vi "Orca Flash Engine.vi"(0 "Notifier Name":string, 11 "Camera ID":string[](array[string])) -> ()   [LabVIEW 2021]
uses:
  Orca Flash Controls/Orca Flash Parameters.ctl
  Orca Flash Controls/Orca Flash Parameter List.ctl
  Orca Flash Controls/Orca Flash ROI.ctl
  Orca Flash Controls/Orca Flash Notifier Element.ctl
  Orca Flash Controls/Orca Flash Actions.ctl
  <vilib>/vision/Image Controls.llb/IMAQ Image.ctl
  Camera Controls/Camera IMAQ Key Info.ctl
panel:
  out "bead collection":bool
  in  "Orca Flash ROI":T1
  in  "Use Display Module":bool
  in  "Sensor Mode":enum32{"Area", "Progressive"}(radio)
  in  "Number of lines":dbl=8.0
  in  "Internal Line Interval Setpoint":dbl=0.001
  in  "Get Parameter":bool
  in  "Set Parameter":bool
  in  "Get ROI":bool
  in  "Set ROI":bool
  in  "sCMOS Parameter":T2={"Value"=0.0, "Orca Flash Parameters"=2049184} {"Orca Flash Parameters" items=["SENSOR MODE"=4212128, "READOUT SPEED"=4211872, "READOUT DIRECTION"=4211904, "TRIGGER GLOBAL EXPOSURE"=2049680, "TRIGGER DELAY"=1066480, "SYNC READOUT SYSTEM BLANK"=1066528, "SENSOR COOLER"=2115248, "SENSOR COOLER STATUS"=2115280, "EXPOSURE TIME"=2049184, "DEFECT CORRECT MODE"=4670368, "BINNING"=4215968, "INTERNAL FRAME RATE"=4225952, "INTERNAL FRAME INTERVAL"=4225968, "INTERNAL LINE SPEED"=4226000, "INTERNAL LINE INTERVAL"=4226016, "IMAGE PIXEL TYPE"=4343296, "NUMBER OF OUTPUT TRIGGER CONNECTOR"=1852320, "OUTPUT TRIGGER SOURCE[0]"=1852576, "OUTPUT TRIGGER SOURCE[1]"=1852832, "OUTPUT TRIGGER SOURCE[2]"=1853088, "OUTPUT TRIGGER POLARITY[0]"=1852592, "OUTPUT TRIGGER POLARITY[1]"=1852848, "OUTPUT TRIGGER POLARITY[2]"=1853104, "OUTPUT TRIGGER ACTIVE[0]"=1852608, "OUTPUT TRIGGER ACTIVE[1]"=1852864, "OUTPUT TRIGGER ACTIVE[2]"=1853120, "OUTPUT TRIGGER DELAY[0]"=1852624, "OUTPUT TRIGGER DELAY[1]"=1852880, "OUTPUT TRIGGER DELAY[2]"=1853136, "OUTPUT TRIGGER PERIOD[0]"=1852640, "OUTPUT TRIGGER PERIOD[1]"=1852896, "OUTPUT TRIGGER PERIOD[2]"=1853152, "OUTPUT TRIGGER KIND[0]"=1852656, "OUTPUT TRIGGER KIND[1]"=1852912, "OUTPUT TRIGGER KIND[2]"=1853168, "OUTPUT TRIGGER PRE HSYNC COUNT"=1852704]}
  in  "# of frames":i32=100
  in  "Path":path
  in  "RECORD":bool
  in  "PREVIEW":bool
  out "Acquisition Loop":i32
  in  "QUIT":bool
  out "Acquisition Frame":i32
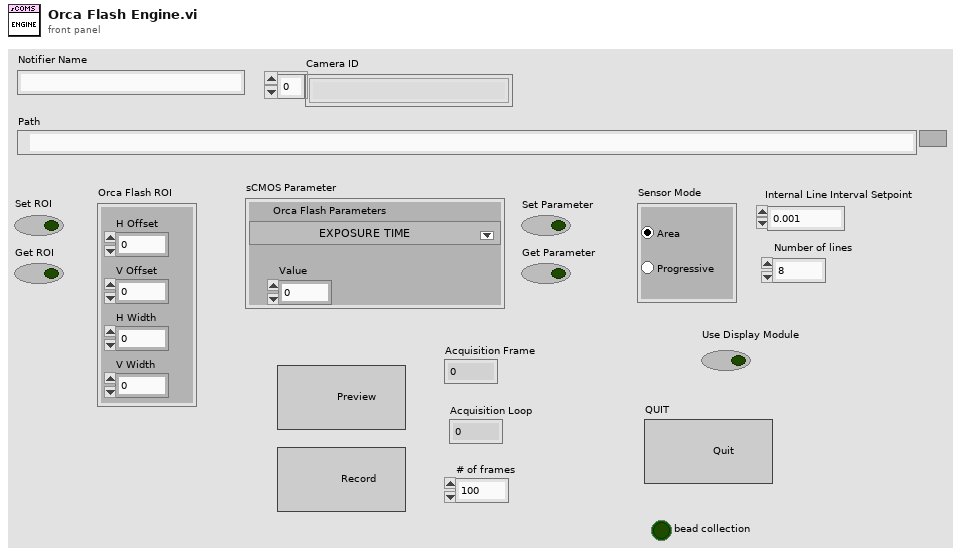
[diagram p1: front panel]
types:
  T1 = typedef "Orca Flash ROI.ctl" = cluster{"H Offset":i32, "V Offset":i32, "H Width":i32, "V Width":i32}
  T2 = typedef "Orca Flash Parameters.ctl" = cluster{"Value":dbl, "Orca Flash Parameters":T3}
  T3 = typedef "Orca Flash Parameter List.ctl" = u32
  T4 = typedef "Camera IMAQ Key Info.ctl" = cluster{"Frame":u32, "Sensor Height":i32, "Sensor Width":i32, "ROI Height":i32, "ROI Width":i32, "ROI Enable?":bool, "Bit per Pixel":u8}
  T5 = typedef "Image Type" = u32
  T6 = typedef "Orca Flash Notifier Element.ctl" = cluster{"Camera Actions":T7, "Received?":bool, "Running?":bool, "sCMOS Parameter":T2, "sCMOS ROI":T1, "Save Path":path, "# of frames":u32, "Image Ref":T8, "Trigger?":bool, "bead collection":bool}
  T7 = typedef "Orca Flash Actions.ctl" = enum16{"IDLE", "PREVIEW", "RECORD", "Send Trigger", "SOFT TRIGGER", "Record Settings", "SETPARAM", "GETPARAM", "SETROI", "GETROI", "PROGRESSIVE MODE", "AREA MODE", "STATUS", "QUIT"}
  T8 = typedef "IMAQ Image.ctl" = refnum<image>
  T9 = enum32{"Invalid", "Standard", "Closed", "Hidden", "Minimized", "Maximized"}
  T10 = cluster{"Horizontal Offset":i32, "Vertical Offset":i32, "Horizontal Size":i32, "Vertical Size":i32}
  T11 = typedef "LVMinMaxIncTypeDef.ctl" = cluster{"Minimum":dbl, "Maximum":dbl, "Increment":dbl}
  T12 = cluster{"H Offset":cluster{"Value":i32, "Limits":T11}, "V Offset":cluster{"Value":i32, "Limits":T11}, "H Size":cluster{"Value":i32, "Limits":T11}, "V Size":cluster{"Value":i32, "Limits":T11}}
  T13 = cluster{"Input Trigger Mode":u32, "Input Trigger Polarity":u32, "Times":u32, "Delay":dbl}
  T14 = cluster{"Output Trigger Period":dbl, "Delay":dbl, "Source":u32}
  T15 = cluster{"Output Trigger Mode":u32, "Output Trigger Polarity":u32}
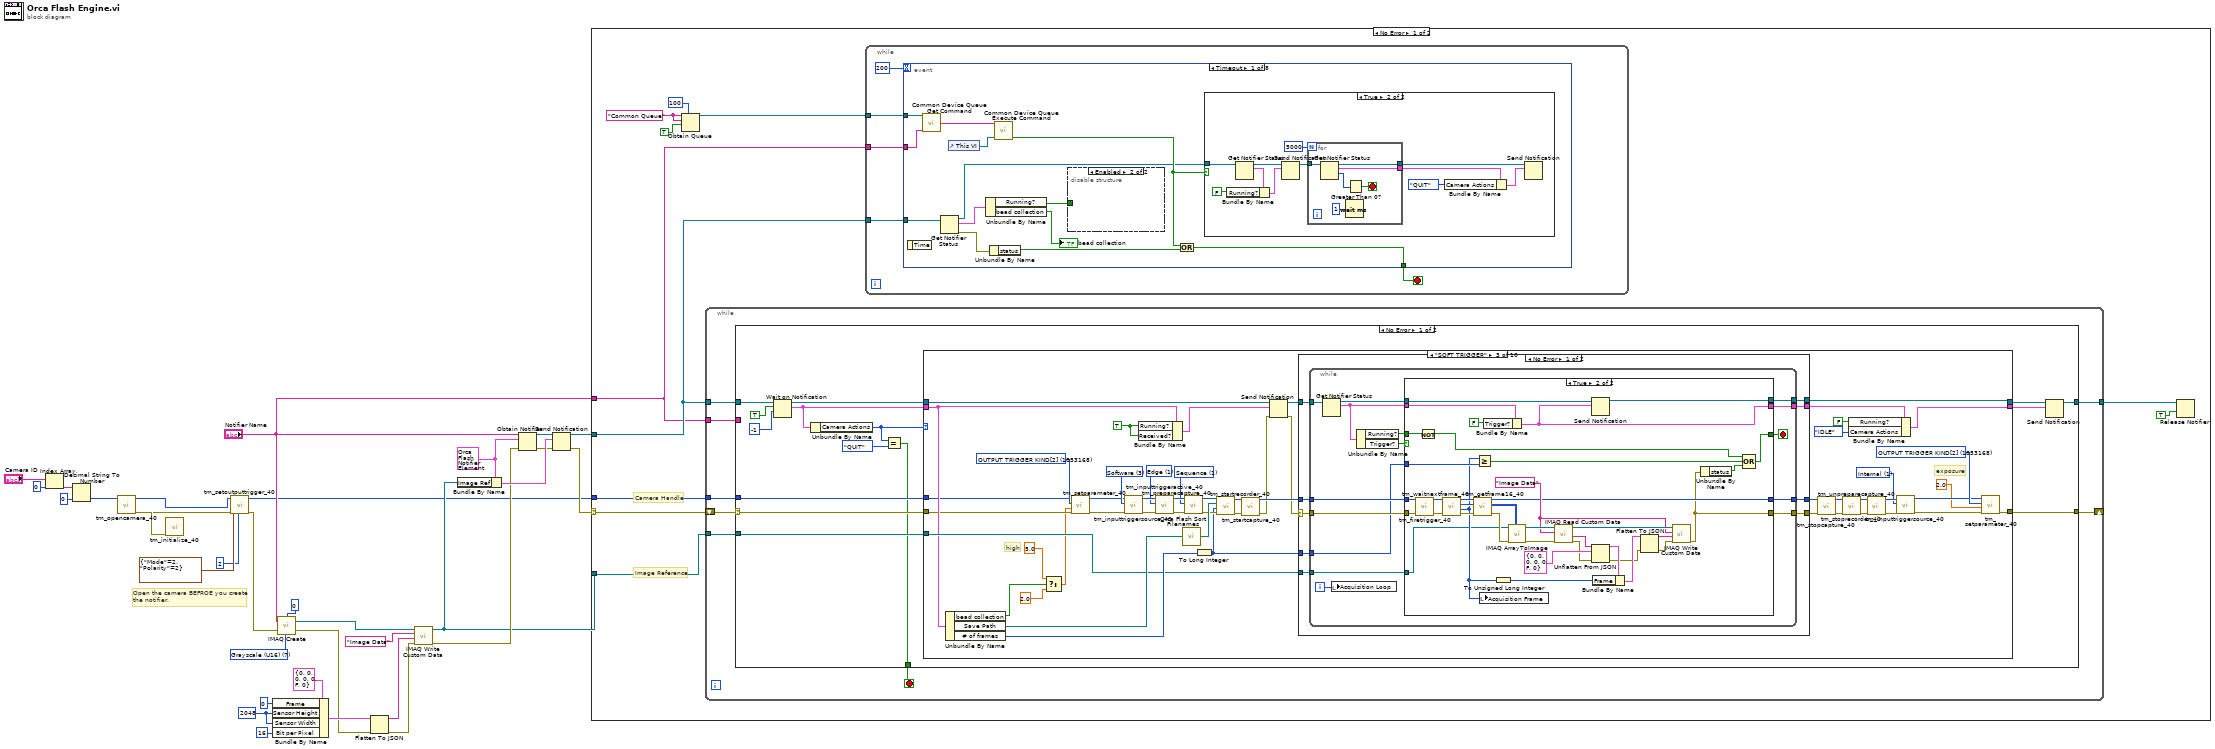
[diagram p0: block diagram]
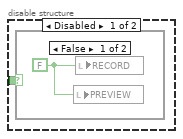
[diagram p2: hidden frame]
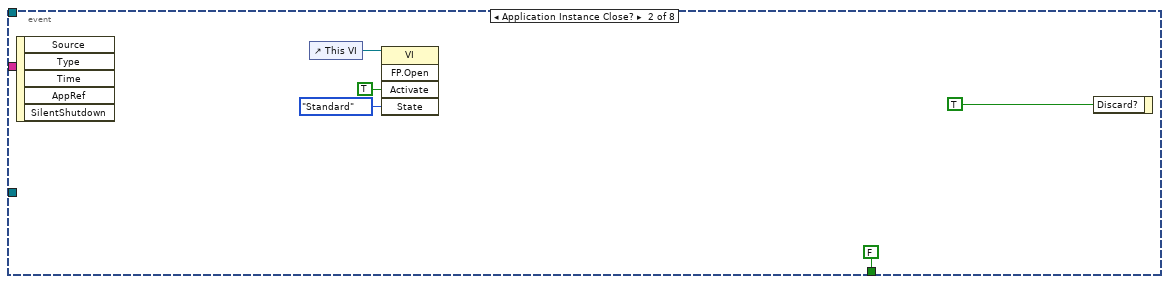
[diagram p5: hidden frame]
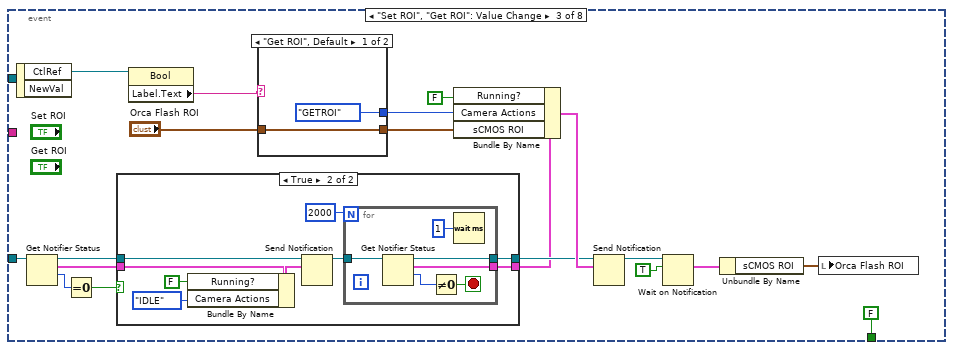
[diagram p6: hidden frame]
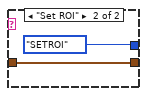
[diagram p8: hidden frame]
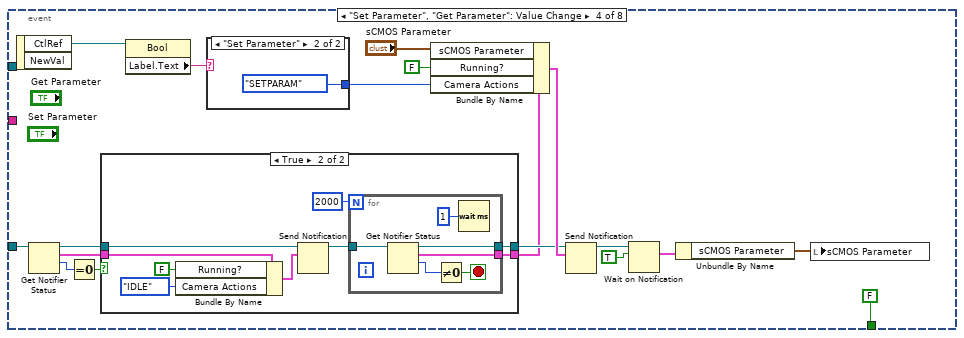
[diagram p9: hidden frame]
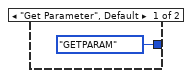
[diagram p11: hidden frame]
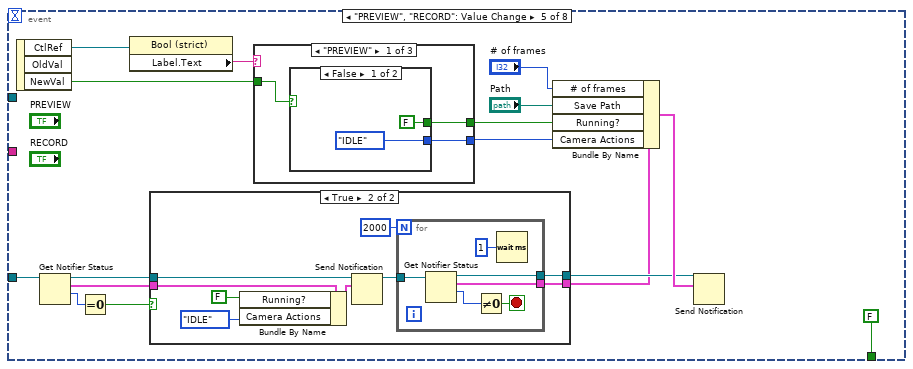
[diagram p12: hidden frame]
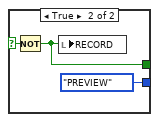
[diagram p13: hidden frame]
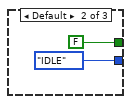
[diagram p14: hidden frame]
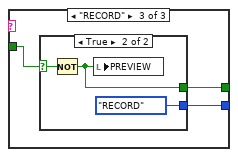
[diagram p15: hidden frame]
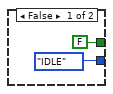
[diagram p16: hidden frame]
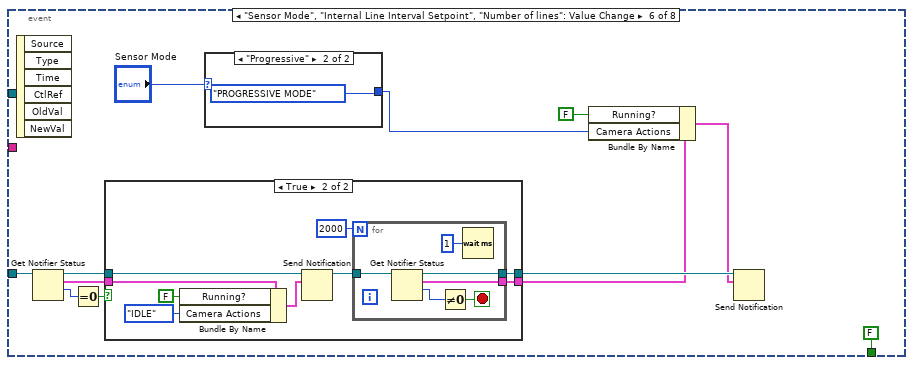
[diagram p18: hidden frame]
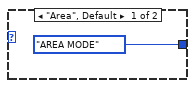
[diagram p19: hidden frame]
diagram:
  w18 = 2048 ("Sensor Height")
  w14 = T5 7 items=["Grayscale (U8)", "Grayscale (I16)", "Grayscale (SGL)", "Complex (CSG)", "RGB (U32)", "HSL (U32)", "RGB (U64)", "Grayscale (U16)"] ("Image Type")
  w28 = T6 {"Camera Actions"=enum."IDLE", "Received?"=FALSE, "Running?"=FALSE, "sCMOS Parameter"={"Value"=0.0, "Orca Flash Parameters"=0}, "sCMOS ROI"={"H Offset"=0, "V Offset"=0, "H Width"=0, "V Width"=0}, "Save Path"=path "", "# of frames"=1, "Image Ref"=refnum, "Trigger?"=FALSE, "bead collection"=FALSE} ("Camera Cluster")
  # "Open the camera BEFROE you create\nthe notifier."
  n1 = Index Array(array="Camera ID", index=0) -> (element=w31:string)
  n2 = Decimal String To Number(string=w31, default (0L)=u32 0 ("default (0 I32)")) -> (number=w24:u32)  [unwired: 1 in, 1 out]
  n3 = call <userlib>:"tm_initialize_40.vi"() -> ("error out"=w25:errorcluster)  [unwired: 8 in, 3 out]
  n4 = call <userlib>:"tm_opencamera_40.vi"("error in (no error)"=w25, "Camera Index"=w24) -> ("error out"=w4:errorcluster, "Handle out"=w3:u32)  [unwired: 7 in, 1 out]
  n5 = call <userlib>:"tm_setoutputtrigger_40.vi"("Port"=2, "error in (no error)"=w4, "Type"=cluster{"Mode":u32, "Polarity":u32} {"Mode"=2, "Polarity"=2}, "Handle in"=w3) -> ("error out"=w6:errorcluster, "Handle out"=w5:u32)  [unwired: 6 in]
  n6 = Bundle By Name(cluster=T4 {"Frame"=0, "Sensor Height"=0, "Sensor Width"=0, "ROI Height"=0, "ROI Width"=0, "ROI Enable?"=FALSE, "Bit per Pixel"=0} ("Camera IMAQ Key Info"), "Frame"=u32 0, "Sensor Height"=w18, "Sensor Width"=w18, "Bit per Pixel"=u8 16) -> (w21:T4)
  n7 = call "IMAQ Create"("Border Size"=0, "Image Name"="Notifier Name", "Image Type"=w14, "error in (no error)"=w6) -> ("New Image"=w16:T8, "error out"=w13:errorcluster)  [unwired: 1 in]
  n8 = Flatten To JSON(anything=w21, error in (no error)=w13) -> (JSON string=w22:string, 11:w12:errorcluster)  [unwired: 1 in]
  n9 = call "IMAQ Write Custom Data"("error in (no error)"=w12, "Custom Data In"=w22, "Key"="Image Data", "Image"=w16) -> ("error out"=w11:errorcluster, "Image Out"=w8:T8)  [unwired: 6 in]
  n10 = Bundle By Name(cluster=w28, "Image Ref"=w8) -> (w29:T6)
  n11 = Obtain Notifier(name (unnamed)="Notifier Name", notification data type=w28, error in (no error)=w11) -> (notifier out=w27:refnum<notifier>, error out=w26:errorcluster)  [unwired: 1 in, 1 out]
  n12 = Send Notification(notification=w29, notifier=w27, error in (no error)=w26) -> (notifier out=w10:refnum<notifier>, error out=w7:errorcluster)
  n13 = case shown="No Error" w7 {
    selector: w7 -> [w39 w760]
    tunnel: w10 -> [w37 w753]
    tunnel: "Notifier Name" -> [w34 w750]
    tunnel: w8 -> [w40 _]
    tunnel: w5 -> [w38 _]
    frame No Error {
      w44 = "Common Queue" ("Unique Notifier Name")
      # "Image Reference"
      # "Camera Handle"
      n14 = Obtain Queue(max queue size (-1, unlimited)=100, name (unnamed)=w44, element data type=w44, create if not found? (T)=TRUE) -> (queue out=w41:refnum<queue>)  [unwired: 1 in, 2 out]
      n15 = while {
        tunnel: w37 -> [w319]
        tunnel: w40 -> [w318]
        shift-right: [w316] -> _
        shift-left: w39 -> [w315]
        tunnel: w38 -> [w317]
        tunnel: [w314] -> w35
        tunnel: w34 -> [w312]
        stop <- w313 stop-if-true
        n16 = case shown="No Error" w315 {
          selector: w315 -> [w324 w741]
          tunnel: w319 -> [w334 w749]
          tunnel: w318 -> [w333 _]
          tunnel: [w323 w749] -> w314
          tunnel: w317 -> [w326 _]
          tunnel: [w325 errorcluster {"status"=FALSE, "code"=0, "source"=""} ("error out")] -> w316
          tunnel: [w320 FALSE] -> w313
          tunnel: w312 -> [_ w740]
          frame No Error {
            n17 = Wait on Notification(notifier=w334, ignore previous (F)=TRUE, timeout in ms (-1)=-1) -> (notifier out=w329:refnum<notifier>, notification=w328:T6)  [unwired: 1 in, 2 out]
            n18 = Unbundle By Name(w328) -> ("Camera Actions"=w322:T7)
            n19 = Equal?(x=w322, y=Orca_Flash_Actions."QUIT") -> (x = y?=w320:bool)
            n20 = case shown="\"SOFT TRIGGER\"" w322 {
              selector: w322 -> [_ w358 _ _ _ _ _ _ _ _]
              tunnel: w326 -> [_ w353 w466 w581 w597 w610 w644 w655 w676 w730]
              tunnel: w324 -> [w339 w350 w465 w582 w596 w609 w643 w654 w675 w729]
              tunnel: [w339 w344 w459 w580 w592 w608 w636 w653 w663 w719] -> w325
              tunnel: w329 -> [w338 w384 w472 w588 w601 w611 w645 w660 w690 w739]
              tunnel: w333 -> [_ w355 w477 w583 _ _ w612 _ _ _]
              tunnel: w328 -> [w336 w375 w473 w586 w595 w606 w639 w657 w687 w726]
              tunnel: [w338 w376 w476 w588 w601 w611 w645 w660 w690 w739] -> w330
              tunnel: [w335 w371 w478 w585 w600 w602 w638 w656 w686 w725] -> w327
              frame "IDLE", Default {
                w337 = FALSE ("Running?")
                n21 = Bundle By Name(cluster=w336, "Received?"=w337, "Running?"=w337) -> (w335:T6)
              }
              frame "PREVIEW", "RECORD" {
                w348 = T3 1853168 items=["SENSOR MODE"=4212128, "READOUT SPEED"=4211872, "READOUT DIRECTION"=4211904, "TRIGGER GLOBAL EXPOSURE"=2049680, "TRIGGER DELAY"=1066480, "SYNC READOUT SYSTEM BLANK"=1066528, "SENSOR COOLER"=2115248, "SENSOR COOLER STATUS"=2115280, "EXPOSURE TIME"=2049184, "DEFECT CORRECT MODE"=4670368, "BINNING"=4215968, "INTERNAL FRAME RATE"=4225952, "INTERNAL FRAME INTERVAL"=4225968, "INTERNAL LINE SPEED"=4226000, "INTERNAL LINE INTERVAL"=4226016, "IMAGE PIXEL TYPE"=4343296, "NUMBER OF OUTPUT TRIGGER CONNECTOR"=1852320, "OUTPUT TRIGGER SOURCE[0]"=1852576, "OUTPUT TRIGGER SOURCE[1]"=1852832, "OUTPUT TRIGGER SOURCE[2]"=1853088, "OUTPUT TRIGGER POLARITY[0]"=1852592, "OUTPUT TRIGGER POLARITY[1]"=1852848, "OUTPUT TRIGGER POLARITY[2]"=1853104, "OUTPUT TRIGGER ACTIVE[0]"=1852608, "OUTPUT TRIGGER ACTIVE[1]"=1852864, "OUTPUT TRIGGER ACTIVE[2]"=1853120, "OUTPUT TRIGGER DELAY[0]"=1852624, "OUTPUT TRIGGER DELAY[1]"=1852880, "OUTPUT TRIGGER DELAY[2]"=1853136, "OUTPUT TRIGGER PERIOD[0]"=1852640, "OUTPUT TRIGGER PERIOD[1]"=1852896, "OUTPUT TRIGGER PERIOD[2]"=1853152, "OUTPUT TRIGGER KIND[0]"=1852656, "OUTPUT TRIGGER KIND[1]"=1852912, "OUTPUT TRIGGER KIND[2]"=1853168, "OUTPUT TRIGGER PRE HSYNC COUNT"=1852704] ("sCMOS Parameter.Orca Flash Parameters")
                w351 = T3 1853168 items=["SENSOR MODE"=4212128, "READOUT SPEED"=4211872, "READOUT DIRECTION"=4211904, "TRIGGER GLOBAL EXPOSURE"=2049680, "TRIGGER DELAY"=1066480, "SYNC READOUT SYSTEM BLANK"=1066528, "SENSOR COOLER"=2115248, "SENSOR COOLER STATUS"=2115280, "EXPOSURE TIME"=2049184, "DEFECT CORRECT MODE"=4670368, "BINNING"=4215968, "INTERNAL FRAME RATE"=4225952, "INTERNAL FRAME INTERVAL"=4225968, "INTERNAL LINE SPEED"=4226000, "INTERNAL LINE INTERVAL"=4226016, "IMAGE PIXEL TYPE"=4343296, "NUMBER OF OUTPUT TRIGGER CONNECTOR"=1852320, "OUTPUT TRIGGER SOURCE[0]"=1852576, "OUTPUT TRIGGER SOURCE[1]"=1852832, "OUTPUT TRIGGER SOURCE[2]"=1853088, "OUTPUT TRIGGER POLARITY[0]"=1852592, "OUTPUT TRIGGER POLARITY[1]"=1852848, "OUTPUT TRIGGER POLARITY[2]"=1853104, "OUTPUT TRIGGER ACTIVE[0]"=1852608, "OUTPUT TRIGGER ACTIVE[1]"=1852864, "OUTPUT TRIGGER ACTIVE[2]"=1853120, "OUTPUT TRIGGER DELAY[0]"=1852624, "OUTPUT TRIGGER DELAY[1]"=1852880, "OUTPUT TRIGGER DELAY[2]"=1853136, "OUTPUT TRIGGER PERIOD[0]"=1852640, "OUTPUT TRIGGER PERIOD[1]"=1852896, "OUTPUT TRIGGER PERIOD[2]"=1853152, "OUTPUT TRIGGER KIND[0]"=1852656, "OUTPUT TRIGGER KIND[1]"=1852912, "OUTPUT TRIGGER KIND[2]"=1853168, "OUTPUT TRIGGER PRE HSYNC COUNT"=1852704] ("sCMOS Parameter.Orca Flash Parameters")
                w356 = TRUE ("Running?")
                w381 = 1 items=["Snap", "Sequence"] ("Capture mode")
                # "exposure"
                # "high"
                n22 = Unbundle By Name(w375) -> ("bead collection"=w340:bool, "# of frames"=w364:u32, "Save Path"=w354:path)
                n23 = Select(t=5.0 ("Value in"), s=w340, f=2.0 ("Value in")) -> (s? t:f=w341:dbl)
                n24 = call <userlib>:"tm_setparameter_40.vi"("error in (no error)"=w350, "Value in"=w341, "Parameter"=w351, "Handle in"=w353) -> ("error out"=w349:errorcluster, "Handle out"=w352:u32)  [unwired: 6 in]
                n25 = Equal?(x=w358, y=Orca_Flash_Actions."RECORD") -> (x = y?=w357:bool)
                n26 = call <userlib>:"tm_preparecapture_40.vi"("error in (no error)"=w349, "Capture mode"=w381, "Handle in"=w352) -> ("error out"=w383:errorcluster, "Handle out"=w382:u32)  [unwired: 5 in, 2 out]
                n27 = To Long Integer(number=w364) -> (32bit integer=w362:i32)
                n28 = case shown="True" w357 {
                  tunnel: w383 -> [w386 w393]
                  tunnel: w382 -> [w385 w392]
                  tunnel: [w385 w391] -> w370
                  tunnel: [w386 w390] -> w368
                  tunnel: w362 -> [_ w389]
                  tunnel: w354 -> [_ w388]
                  frame False {
                  }
                  frame True {
                    n29 = call "Orca Flash Sort Filenames.vi"("Requested File Path"=w388) -> ("Resulting File Path"=w387:path)  [unwired: 14 in]
                    n30 = call <userlib>:"tm_startrecorder_40.vi"("error in (no error)"=w393, "frames"=w389, "File"=w387, "Handle in"=w392) -> ("error out"=w390:errorcluster, "Handle out"=w391:u32)  [unwired: 6 in]
                  }
                }
                n31 = Bundle By Name(cluster=w375, "Running?"=w356, "Received?"=w356) -> (w374:T6)
                n32 = call <userlib>:"tm_startcapture_40.vi"("error in (no error)"=w368, "Handle in"=w370) -> ("error out"=w361:errorcluster, "Handle out"=w369:u32)  [unwired: 8 in]
                n33 = Send Notification(notification=w374, notifier=w384, error in (no error)=w361) -> (notifier out=w377:refnum<notifier>, error out=w360:errorcluster)
                n34 = case shown="No Error" w360 {
                  selector: w360 -> [w401 w451]
                  tunnel: [w409 w452] -> w380
                  tunnel: w377 -> [w408 w453]
                  tunnel: w355 -> [w407 _]
                  tunnel: [w406 w450] -> w376
                  tunnel: [w405 w449] -> w373
                  tunnel: w369 -> [w404 w452]
                  tunnel: [w403 w451] -> w367
                  tunnel: w362 -> [w402 _]
                  tunnel: w357 -> [w400 _]
                  frame No Error {
                    n35 = while {
                      tunnel: w402 -> [w437]
                      tunnel: w408 -> [w440]
                      tunnel: [w439] -> w406
                      tunnel: w407 -> [w436]
                      tunnel: [w434] -> w405
                      tunnel: w401 -> [w443]
                      tunnel: [w411] -> w403
                      tunnel: w404 -> [w444]
                      tunnel: [w432] -> w409
                      tunnel: w400 -> [w410]
                      i -> [w438]
                      stop <- w441 stop-if-true
                      w417 = "Image Data" ("Key")
                      n36 = call <userlib>:"tm_waitnextframe_40.vi"("error in (no error)"=w443, "Handle in"=w444) -> ("error out"=w428:errorcluster, "Frame Count"=w426:i32, "Frame Index"=w431:i32, "Handle out"=w442:u32)  [unwired: 6 in]
                      "Acquisition Frame" <- w426
                      n37 = call <userlib>:"tm_getframe16_40.vi"("error in (no error)"=w428, "Frame Index"=w431, "Handle in"=w442) -> ("error out"=w416:errorcluster, "Data"=w427:u16[][], "Handle out"=w432:u32)  [unwired: 5 in, 1 out]
                      n38 = case shown="True" w410 {
                        selector: w410 -> [w445 _]
                        tunnel: w437 -> [_ w448]
                        tunnel: [w445 w447] -> w429
                        tunnel: w426 -> [_ w446]
                        frame False {
                        }
                        frame True {
                          n39 = Greater Or Equal?(x=w446, y=w448) -> (x >= y?=w447:bool)
                        }
                      }
                      n40 = To Unsigned Long Integer(number=w426) -> (unsigned 32bit integer=w420:u32)
                      n41 = call "IMAQ ArrayToImage"("Image Pixels (U16)"=w427, "error in (no error)"=w416, "Image"=w436) -> ("error out"=w415:errorcluster, "Image Out"=w425:T8)  [unwired: 7 in]
                      n42 = call "IMAQ Read Custom Data"("error in (no error)"=w415, "Key"=w417, "Image"=w425) -> ("error out"=w414:errorcluster, "Custom Data Out"=w422:string, "Image (duplicate)"=w424:T8)  [unwired: 6 in]
                      n43 = Unflatten From JSON(JSON string=w422, type and defaults=T4 {"Frame"=0, "Sensor Height"=0, "Sensor Width"=0, "ROI Height"=0, "ROI Width"=0, "ROI Enable?"=FALSE, "Bit per Pixel"=0} ("Camera IMAQ Key Info"), error in (no error)=w414) -> (value=w421:T4, error out=w413:errorcluster)  [unwired: 4 in]
                      n44 = Bundle By Name(cluster=w421, "Frame"=w420) -> (w419:T4)
                      n45 = Get Notifier Status(notifier=w440) -> (notifier out=w439:refnum<notifier>, current notification=w434:T6)  [unwired: 1 in, 3 out]
                      n46 = Flatten To JSON(anything=w419, error in (no error)=w413) -> (JSON string=w418:string, 11:w412:errorcluster)  [unwired: 1 in]
                      n47 = Unbundle By Name(w434) -> ("Running?"=w435:bool)
                      n48 = call "IMAQ Write Custom Data"("error in (no error)"=w412, "Custom Data In"=w418, "Key"=w417, "Image"=w424) -> ("error out"=w411:errorcluster)  [unwired: 6 in, 1 out]
                      n49 = Unbundle By Name(w411) -> ("status"=w430:bool)
                      n50 = Not(x=w435) -> (.not. x?=w433:bool)
                      n51 = Compound Arithmetic op=OR(w433, w429, w430) -> (w441:bool)
                      "Acquisition Loop" <- w438
                    }
                  }
                  frame Error {
                    n52 = Get Notifier Status(notifier=w453) -> (notifier out=w450:refnum<notifier>, current notification=w449:T6)  [unwired: 1 in, 3 out]
                  }
                }
                n53 = call <userlib>:"tm_stopcapture_40.vi"("error in (no error)"=w367, "Handle in"=w380) -> ("error out"=w366:errorcluster, "Handle out"=w379:u32)  [unwired: 8 in]
                n54 = case shown="True" w357 {
                  tunnel: w379 -> [w395 w399]
                  tunnel: [w395 w398] -> w378
                  tunnel: w366 -> [w394 w397]
                  tunnel: [w394 w396] -> w365
                  frame False {
                  }
                  frame True {
                    n55 = call <userlib>:"tm_stoprecorder_40.vi"("error in (no error)"=w397, "Handle in"=w399) -> ("error out"=w396:errorcluster, "Handle out"=w398:u32)  [unwired: 8 in]
                  }
                }
                n56 = Bundle By Name(cluster=w373, "Running?"=FALSE, "Camera Actions"=Orca_Flash_Actions."IDLE") -> (w371:T6)
                n57 = call <userlib>:"tm_unpreparecapture_40.vi"("error in (no error)"=w365, "Handle in"=w378) -> ("error out"=w345:errorcluster, "Handle out"=w346:u32)  [unwired: 8 in]
                n58 = call <userlib>:"tm_setparameter_40.vi"("error in (no error)"=w345, "Value in"=2.0, "Parameter"=w348, "Handle in"=w346) -> ("error out"=w344:errorcluster)  [unwired: 6 in, 1 out]
              }
              frame "SOFT TRIGGER" {
                w462 = T3 1853168 items=["SENSOR MODE"=4212128, "READOUT SPEED"=4211872, "READOUT DIRECTION"=4211904, "TRIGGER GLOBAL EXPOSURE"=2049680, "TRIGGER DELAY"=1066480, "SYNC READOUT SYSTEM BLANK"=1066528, "SENSOR COOLER"=2115248, "SENSOR COOLER STATUS"=2115280, "EXPOSURE TIME"=2049184, "DEFECT CORRECT MODE"=4670368, "BINNING"=4215968, "INTERNAL FRAME RATE"=4225952, "INTERNAL FRAME INTERVAL"=4225968, "INTERNAL LINE SPEED"=4226000, "INTERNAL LINE INTERVAL"=4226016, "IMAGE PIXEL TYPE"=4343296, "NUMBER OF OUTPUT TRIGGER CONNECTOR"=1852320, "OUTPUT TRIGGER SOURCE[0]"=1852576, "OUTPUT TRIGGER SOURCE[1]"=1852832, "OUTPUT TRIGGER SOURCE[2]"=1853088, "OUTPUT TRIGGER POLARITY[0]"=1852592, "OUTPUT TRIGGER POLARITY[1]"=1852848, "OUTPUT TRIGGER POLARITY[2]"=1853104, "OUTPUT TRIGGER ACTIVE[0]"=1852608, "OUTPUT TRIGGER ACTIVE[1]"=1852864, "OUTPUT TRIGGER ACTIVE[2]"=1853120, "OUTPUT TRIGGER DELAY[0]"=1852624, "OUTPUT TRIGGER DELAY[1]"=1852880, "OUTPUT TRIGGER DELAY[2]"=1853136, "OUTPUT TRIGGER PERIOD[0]"=1852640, "OUTPUT TRIGGER PERIOD[1]"=1852896, "OUTPUT TRIGGER PERIOD[2]"=1853152, "OUTPUT TRIGGER KIND[0]"=1852656, "OUTPUT TRIGGER KIND[1]"=1852912, "OUTPUT TRIGGER KIND[2]"=1853168, "OUTPUT TRIGGER PRE HSYNC COUNT"=1852704] ("sCMOS Parameter.Orca Flash Parameters")
                w467 = T3 1853168 items=["SENSOR MODE"=4212128, "READOUT SPEED"=4211872, "READOUT DIRECTION"=4211904, "TRIGGER GLOBAL EXPOSURE"=2049680, "TRIGGER DELAY"=1066480, "SYNC READOUT SYSTEM BLANK"=1066528, "SENSOR COOLER"=2115248, "SENSOR COOLER STATUS"=2115280, "EXPOSURE TIME"=2049184, "DEFECT CORRECT MODE"=4670368, "BINNING"=4215968, "INTERNAL FRAME RATE"=4225952, "INTERNAL FRAME INTERVAL"=4225968, "INTERNAL LINE SPEED"=4226000, "INTERNAL LINE INTERVAL"=4226016, "IMAGE PIXEL TYPE"=4343296, "NUMBER OF OUTPUT TRIGGER CONNECTOR"=1852320, "OUTPUT TRIGGER SOURCE[0]"=1852576, "OUTPUT TRIGGER SOURCE[1]"=1852832, "OUTPUT TRIGGER SOURCE[2]"=1853088, "OUTPUT TRIGGER POLARITY[0]"=1852592, "OUTPUT TRIGGER POLARITY[1]"=1852848, "OUTPUT TRIGGER POLARITY[2]"=1853104, "OUTPUT TRIGGER ACTIVE[0]"=1852608, "OUTPUT TRIGGER ACTIVE[1]"=1852864, "OUTPUT TRIGGER ACTIVE[2]"=1853120, "OUTPUT TRIGGER DELAY[0]"=1852624, "OUTPUT TRIGGER DELAY[1]"=1852880, "OUTPUT TRIGGER DELAY[2]"=1853136, "OUTPUT TRIGGER PERIOD[0]"=1852640, "OUTPUT TRIGGER PERIOD[1]"=1852896, "OUTPUT TRIGGER PERIOD[2]"=1853152, "OUTPUT TRIGGER KIND[0]"=1852656, "OUTPUT TRIGGER KIND[1]"=1852912, "OUTPUT TRIGGER KIND[2]"=1853168, "OUTPUT TRIGGER PRE HSYNC COUNT"=1852704] ("sCMOS Parameter.Orca Flash Parameters")
                w474 = TRUE ("Running?")
                w481 = 1 items=["Internal"=1, "External"=2, "Software"=3, "Master Pulse"=4] ("Source")
                w500 = 1 items=["Snap", "Sequence"] ("Capture mode")
                w503 = 1 items=["Edge"=1, "Level"=2, "Sync Readout"=3, "Point"=4] ("Active")
                w505 = 3 items=["Internal"=1, "External"=2, "Software"=3, "Master Pulse"=4] ("Source")
                # "high"
                # "exposure"
                n59 = Unbundle By Name(w473) -> ("bead collection"=w454:bool, "Save Path"=w498:path, "# of frames"=w497:u32)
                n60 = Select(t=5.0 ("Value in"), s=w454, f=2.0 ("Value in")) -> (s? t:f=w455:dbl)
                n61 = call <userlib>:"tm_setparameter_40.vi"("error in (no error)"=w465, "Value in"=w455, "Parameter"=w467, "Handle in"=w466) -> ("error out"=w463:errorcluster, "Handle out"=w464:u32)  [unwired: 6 in]
                n62 = call <userlib>:"tm_inputtriggersource_40.vi"("error in (no error)"=w463, "Source"=w505, "Handle in"=w464) -> ("error out"=w495:errorcluster, "Handle out"=w504:u32)  [unwired: 7 in]
                n63 = Bundle By Name(cluster=w473, "Running?"=w474, "Received?"=w474) -> (w470:T6)
                n64 = call <userlib>:"tm_inputtriggeractive_40.vi"("error in (no error)"=w495, "Active"=w503, "Handle in"=w504) -> ("error out"=w494:errorcluster, "Handle out"=w502:u32)  [unwired: 7 in]
                n65 = call "Orca Flash Sort Filenames.vi"("Requested File Path"=w498) -> ("Resulting File Path"=w499:path)  [unwired: 14 in]
                n66 = call <userlib>:"tm_preparecapture_40.vi"("error in (no error)"=w494, "Capture mode"=w500, "Handle in"=w502) -> ("error out"=w493:errorcluster, "Handle out"=w501:u32)  [unwired: 5 in, 2 out]
                n67 = To Long Integer(number=w497) -> (32bit integer=w490:i32)
                n68 = call <userlib>:"tm_startrecorder_40.vi"("error in (no error)"=w493, "frames"=w490, "File"=w499, "Handle in"=w501) -> ("error out"=w492:errorcluster, "Handle out"=w496:u32)  [unwired: 6 in]
                n69 = call <userlib>:"tm_startcapture_40.vi"("error in (no error)"=w492, "Handle in"=w496) -> ("error out"=w469:errorcluster, "Handle out"=w491:u32)  [unwired: 8 in]
                n70 = Send Notification(notification=w470, notifier=w472, error in (no error)=w469) -> (notifier out=w471:refnum<notifier>, error out=w468:errorcluster)
                n71 = case shown="No Error" w468 {
                  selector: w468 -> [w506 w575]
                  tunnel: w491 -> [w514 w576]
                  tunnel: w490 -> [w513 _]
                  tunnel: [w512 w576] -> w489
                  tunnel: [w511 w575] -> w488
                  tunnel: w477 -> [w510 _]
                  tunnel: [w509 w577] -> w476
                  tunnel: [w508 w578] -> w475
                  tunnel: w471 -> [w507 w579]
                  frame No Error {
                    n72 = while {
                      tunnel: w514 -> [w528]
                      tunnel: w506 -> [w527]
                      tunnel: w507 -> [w521]
                      tunnel: w513 -> [w526]
                      tunnel: [w523] -> w512
                      tunnel: [w522] -> w511
                      tunnel: w510 -> [w519]
                      tunnel: [w516] -> w509
                      tunnel: [w515] -> w508
                      i -> [w520]
                      stop <- w524 stop-if-true
                      n73 = Get Notifier Status(notifier=w521) -> (notifier out=w517:refnum<notifier>, current notification=w518:T6)  [unwired: 1 in, 3 out]
                      n74 = local write "Acquisition Loop"(w520) -> ()
                      n75 = Unbundle By Name(w518) -> ("Running?"=w525:bool, "Trigger?"=w529:bool)
                      n76 = case shown="True" w529 {
                        tunnel: w528 -> [w533 w574]
                        tunnel: w527 -> [w532 w573]
                        tunnel: w526 -> [_ w552]
                        tunnel: w525 -> [w537 w551]
                        tunnel: [w536 w547] -> w524
                        tunnel: [w533 w546] -> w523
                        tunnel: [w532 w545] -> w522
                        tunnel: w519 -> [_ w543]
                        tunnel: w518 -> [w531 w542]
                        tunnel: w517 -> [w530 w540]
                        tunnel: [w530 w539] -> w516
                        tunnel: [w531 w538] -> w515
                        frame False {
                          n77 = Unbundle By Name(w532) -> ("status"=w534:bool)
                          n78 = Not(x=w537) -> (.not. x?=w535:bool)
                          n79 = Or(x=w535, y=w534) -> (x .or. y?=w536:bool)
                        }
                        frame True {
                          w561 = "Image Data" ("Key")
                          n80 = call <userlib>:"tm_firetrigger_40.vi"("error in (no error)"=w573, "Handle in"=w574) -> ("error out"=w571:errorcluster, "Handle out"=w572:u32)  [unwired: 8 in]
                          n81 = Not(x=w551) -> (.not. x?=w550:bool)
                          n82 = call <userlib>:"tm_waitnextframe_40.vi"("error in (no error)"=w571, "Handle in"=w572) -> ("error out"=w555:errorcluster, "Frame Count"=w544:i32, "Frame Index"=w553:i32, "Handle out"=w554:u32)  [unwired: 6 in]
                          n83 = call <userlib>:"tm_getframe16_40.vi"("error in (no error)"=w555, "Frame Index"=w553, "Handle in"=w554) -> ("error out"=w560:errorcluster, "Data"=w570:u16[][], "Handle out"=w546:u32)  [unwired: 5 in, 1 out]
                          n84 = Greater Or Equal?(x=w544, y=w552) -> (x >= y?=w549:bool)
                          n85 = local write "Acquisition Frame"(w544) -> ()
                          n86 = Bundle By Name(cluster=w542, "Trigger?"=FALSE) -> (w538:T6)
                          n87 = To Unsigned Long Integer(number=w544) -> (unsigned 32bit integer=w564:u32)
                          n88 = call "IMAQ ArrayToImage"("Image Pixels (U16)"=w570, "error in (no error)"=w560, "Image"=w543) -> ("error out"=w559:errorcluster, "Image Out"=w569:T8)  [unwired: 7 in]
                          n89 = call "IMAQ Read Custom Data"("error in (no error)"=w559, "Key"=w561, "Image"=w569) -> ("error out"=w558:errorcluster, "Custom Data Out"=w566:string, "Image (duplicate)"=w568:T8)  [unwired: 6 in]
                          n90 = Send Notification(notification=w538, notifier=w540) -> (notifier out=w539:refnum<notifier>)  [unwired: 1 in, 1 out]
                          n91 = Unflatten From JSON(JSON string=w566, type and defaults=T4 {"Frame"=0, "Sensor Height"=0, "Sensor Width"=0, "ROI Height"=0, "ROI Width"=0, "ROI Enable?"=FALSE, "Bit per Pixel"=0} ("Camera IMAQ Key Info"), error in (no error)=w558) -> (value=w565:T4, error out=w557:errorcluster)  [unwired: 4 in]
                          n92 = Bundle By Name(cluster=w565, "Frame"=w564) -> (w563:T4)
                          n93 = Flatten To JSON(anything=w563, error in (no error)=w557) -> (JSON string=w562:string, 11:w556:errorcluster)  [unwired: 1 in]
                          n94 = call "IMAQ Write Custom Data"("error in (no error)"=w556, "Custom Data In"=w562, "Key"=w561, "Image"=w568) -> ("error out"=w545:errorcluster)  [unwired: 6 in, 1 out]
                          n95 = Unbundle By Name(w545) -> ("status"=w548:bool)
                          n96 = Compound Arithmetic op=OR(w550, w549, w548) -> (w547:bool)
                        }
                      }
                    }
                  }
                  frame Error {
                    n97 = Get Notifier Status(notifier=w579) -> (notifier out=w577:refnum<notifier>, current notification=w578:T6)  [unwired: 1 in, 3 out]
                  }
                }
                n98 = call <userlib>:"tm_stopcapture_40.vi"("error in (no error)"=w488, "Handle in"=w489) -> ("error out"=w486:errorcluster, "Handle out"=w487:u32)  [unwired: 8 in]
                n99 = call <userlib>:"tm_stoprecorder_40.vi"("error in (no error)"=w486, "Handle in"=w487) -> ("error out"=w484:errorcluster, "Handle out"=w485:u32)  [unwired: 8 in]
                n100 = Bundle By Name(cluster=w475, "Running?"=FALSE, "Camera Actions"=Orca_Flash_Actions."IDLE") -> (w478:T6)
                n101 = call <userlib>:"tm_unpreparecapture_40.vi"("error in (no error)"=w484, "Handle in"=w485) -> ("error out"=w482:errorcluster, "Handle out"=w483:u32)  [unwired: 8 in]
                n102 = call <userlib>:"tm_inputtriggersource_40.vi"("error in (no error)"=w482, "Source"=w481, "Handle in"=w483) -> ("error out"=w460:errorcluster, "Handle out"=w461:u32)  [unwired: 7 in]
                n103 = call <userlib>:"tm_setparameter_40.vi"("error in (no error)"=w460, "Value in"=2.0, "Parameter"=w462, "Handle in"=w461) -> ("error out"=w459:errorcluster)  [unwired: 6 in, 1 out]
              }
              frame "QUIT" {
                n104 = call <userlib>:"tm_closecamera_40.vi"("error in (no error)"=w582, "Handle in"=w581) -> ("error out"=w584:errorcluster)  [unwired: 9 in]
                n105 = call "IMAQ Dispose"("Image"=w583) -> ()  [unwired: 5 in, 1 out]
                n106 = Bundle By Name(cluster=w586, "Received?"=TRUE ("Running?")) -> (w585:T6)
                n107 = call <userlib>:"tm_deinitialize_40.vi"("error in (no error)"=w584) -> ("error out"=w580:errorcluster)  [unwired: 10 in]
              }
              frame "SETPARAM" {
                n108 = Unbundle By Name(w595) -> ("sCMOS Parameter.Orca Flash Parameters"=w590:T3, "sCMOS Parameter.Value"=w594:dbl)
                n109 = call <userlib>:"tm_setparameter_40.vi"("error in (no error)"=w596, "Value in"=w594, "Parameter"=w590, "Handle in"=w597) -> ("error out"=w593:errorcluster, "Handle out"=w591:u32)  [unwired: 6 in]
                n110 = call <userlib>:"tm_getparameter_40.vi"("error in (no error)"=w593, "Parameter"=w590, "Handle in"=w591) -> ("error out"=w592:errorcluster, "Value out"=w589:dbl)  [unwired: 6 in, 1 out]
                n111 = Bundle By Name(cluster=w595, "Received?"=TRUE ("Running?"), "Camera Actions"=Orca_Flash_Actions."IDLE", "sCMOS Parameter.Value"=w589) -> (w600:T6)
              }
              frame "GETPARAM" {
                n112 = Unbundle By Name(w606) -> ("sCMOS Parameter.Orca Flash Parameters"=w607:T3)
                n113 = call <userlib>:"tm_getparameter_40.vi"("error in (no error)"=w609, "Parameter"=w607, "Handle in"=w610) -> ("error out"=w608:errorcluster, "Value out"=w603:dbl)  [unwired: 6 in, 1 out]
                n114 = Bundle By Name(cluster=w606, "Received?"=TRUE ("Running?"), "Camera Actions"=Orca_Flash_Actions."IDLE", "sCMOS Parameter.Value"=w603) -> (w602:T6)
              }
              frame "SETROI" {
                w621 = "Image Data" ("Key")
                n115 = Unbundle By Name(w639) -> ("sCMOS ROI.H Offset"=w626:i32, "sCMOS ROI.V Offset"=w627:i32, "sCMOS ROI.H Width"=w628:i32, "sCMOS ROI.V Width"=w629:i32)
                n116 = Bundle By Name(cluster=T10 {"Horizontal Offset"=0, "Vertical Offset"=0, "Horizontal Size"=0, "Vertical Size"=0} ("Sub Region"), "Horizontal Offset"=w626, "Vertical Offset"=w627, "Horizontal Size"=w628, "Vertical Size"=w629) -> (w625:T10)
                n117 = call <userlib>:"tm_setarea_40.vi"("error in (no error)"=w643, "Sub Region"=w625, "Handle in"=w644) -> ("error out"=w637:errorcluster, "Handle out"=w642:u32)  [unwired: 7 in]
                n118 = call <userlib>:"tm_getarea_40.vi"("error in (no error)"=w637, "Handle in"=w642) -> ("error out"=w636:errorcluster, "Sub Region"=w635:T12)  [unwired: 7 in, 1 out]
                n119 = Unbundle By Name(w635) -> ("H Offset.Value"=w633:i32, "V Offset.Value"=w632:i32, "H Size.Value"=w613:i32, "V Size.Value"=w614:i32)
                n120 = Bundle By Name(cluster=T1 {"H Offset"=0, "V Offset"=0, "H Width"=0, "V Width"=0} ("Orca Flash ROI"), "H Offset"=w633, "V Offset"=w632, "H Width"=w613, "V Width"=w614) -> (w631:T1)
                n121 = Bundle By Name(cluster=w639, "Received?"=TRUE ("Running?"), "Camera Actions"=Orca_Flash_Actions."IDLE", "sCMOS ROI"=w631) -> (w638:T6)
                n122 = call "IMAQ Read Custom Data"("Key"=w621, "Image"=w612) -> ("error out"=w622:errorcluster, "Custom Data Out"=w617:string, "Image (duplicate)"=w615:T8)  [unwired: 7 in]
                n123 = Unflatten From JSON(JSON string=w617, type and defaults=T4 {"Frame"=0, "Sensor Height"=0, "Sensor Width"=0, "ROI Height"=0, "ROI Width"=0, "ROI Enable?"=FALSE, "Bit per Pixel"=0} ("Camera IMAQ Key Info"), error in (no error)=w622) -> (value=w618:T4, error out=w623:errorcluster)  [unwired: 4 in]
                n124 = Bundle By Name(cluster=w618, "ROI Width"=w613, "ROI Height"=w614) -> (w619:T4)
                n125 = Flatten To JSON(anything=w619, error in (no error)=w623) -> (JSON string=w620:string, 11:w624:errorcluster)  [unwired: 1 in]
                n126 = call "IMAQ Write Custom Data"("error in (no error)"=w624, "Custom Data In"=w620, "Key"=w621, "Image"=w615) -> ()  [unwired: 6 in, 2 out]
              }
              frame "GETROI" {
                n127 = call <userlib>:"tm_getarea_40.vi"("error in (no error)"=w654, "Handle in"=w655) -> ("error out"=w653:errorcluster, "Sub Region"=w652:T12)  [unwired: 7 in, 1 out]
                n128 = Unbundle By Name(w652) -> ("H Offset.Value"=w647:i32, "V Offset.Value"=w648:i32, "H Size.Value"=w649:i32, "V Size.Value"=w650:i32)
                n129 = Bundle By Name(cluster=T1 {"H Offset"=0, "V Offset"=0, "H Width"=0, "V Width"=0} ("Orca Flash ROI"), "H Offset"=w647, "V Offset"=w648, "H Width"=w649, "V Width"=w650) -> (w646:T1)
                n130 = Bundle By Name(cluster=w657, "Received?"=TRUE ("Running?"), "Camera Actions"=Orca_Flash_Actions."IDLE", "sCMOS ROI"=w646) -> (w656:T6)
              }
              frame "PROGRESSIVE MODE" {
                w662 = u32 2049184 items=["SENSOR MODE"=4212128, "READOUT SPEED"=4211872, "READOUT DIRECTION"=4211904, "TRIGGER GLOBAL EXPOSURE"=2049680, "TRIGGER DELAY"=1066480, "INTERNAL TRIGGER HANDLING"=1066496, "SYNC READOUT SYSTEM BLANK"=1066528, "SENSOR TEMPERATURE"=2115232, "SENSOR COOLER STATUS"=2115280, "EXPOSURE TIME"=2049184, "DEFECT CORRECT MODE"=4670368, "BINNING"=4215968, "INTERNAL LINE SPEED"=4226000, "INTERNAL LINE INTERVAL"=4226016, "NUMBER OF OUTPUT TRIGGER CONNECTOR"=1852320, "OUTPUT TRIGGER SOURCE[0]"=1852576, "OUTPUT TRIGGER SOURCE[1]"=1852832, "OUTPUT TRIGGER SOURCE[2]"=1853088, "OUTPUT TRIGGER POLARITY[0]"=1852592, "OUTPUT TRIGGER POLARITY[1]"=1852848, "OUTPUT TRIGGER POLARITY[2]"=1853104, "OUTPUT TRIGGER ACTIVE[0]"=1852608, "OUTPUT TRIGGER ACTIVE[1]"=1852864, "OUTPUT TRIGGER ACTIVE[2]"=1853120, "OUTPUT TRIGGER DELAY[0]"=1852624, "OUTPUT TRIGGER DELAY[1]"=1852880, "OUTPUT TRIGGER DELAY[2]"=1853136, "OUTPUT TRIGGER PERIOD[0]"=1852640, "OUTPUT TRIGGER PERIOD[1]"=1852896, "OUTPUT TRIGGER PERIOD[2]"=1853152, "OUTPUT TRIGGER KIND[0]"=1852656, "OUTPUT TRIGGER KIND[1]"=1852912, "OUTPUT TRIGGER KIND[2]"=1853168, "OUTPUT TRIGGER BASE SENSOR[0]"=1852672, "OUTPUT TRIGGER BASE SENSOR[1]"=1852928, "OUTPUT TRIGGER BASE SENSOR[2]"=1853184, "OUTPUT TRIGGER PRE HSYNC COUNT"=1852704] ("Parameter")
                w668 = u32 4226016 items=["SENSOR MODE"=4212128, "READOUT SPEED"=4211872, "READOUT DIRECTION"=4211904, "TRIGGER GLOBAL EXPOSURE"=2049680, "TRIGGER DELAY"=1066480, "INTERNAL TRIGGER HANDLING"=1066496, "SYNC READOUT SYSTEM BLANK"=1066528, "SENSOR TEMPERATURE"=2115232, "SENSOR COOLER STATUS"=2115280, "EXPOSURE TIME"=2049184, "DEFECT CORRECT MODE"=4670368, "BINNING"=4215968, "INTERNAL LINE SPEED"=4226000, "INTERNAL LINE INTERVAL"=4226016, "NUMBER OF OUTPUT TRIGGER CONNECTOR"=1852320, "OUTPUT TRIGGER SOURCE[0]"=1852576, "OUTPUT TRIGGER SOURCE[1]"=1852832, "OUTPUT TRIGGER SOURCE[2]"=1853088, "OUTPUT TRIGGER POLARITY[0]"=1852592, "OUTPUT TRIGGER POLARITY[1]"=1852848, "OUTPUT TRIGGER POLARITY[2]"=1853104, "OUTPUT TRIGGER ACTIVE[0]"=1852608, "OUTPUT TRIGGER ACTIVE[1]"=1852864, "OUTPUT TRIGGER ACTIVE[2]"=1853120, "OUTPUT TRIGGER DELAY[0]"=1852624, "OUTPUT TRIGGER DELAY[1]"=1852880, "OUTPUT TRIGGER DELAY[2]"=1853136, "OUTPUT TRIGGER PERIOD[0]"=1852640, "OUTPUT TRIGGER PERIOD[1]"=1852896, "OUTPUT TRIGGER PERIOD[2]"=1853152, "OUTPUT TRIGGER KIND[0]"=1852656, "OUTPUT TRIGGER KIND[1]"=1852912, "OUTPUT TRIGGER KIND[2]"=1853168, "OUTPUT TRIGGER BASE SENSOR[0]"=1852672, "OUTPUT TRIGGER BASE SENSOR[1]"=1852928, "OUTPUT TRIGGER BASE SENSOR[2]"=1853184, "OUTPUT TRIGGER PRE HSYNC COUNT"=1852704] ("Parameter")
                w679 = u32 1 items=["FORWARD"=1, "BACKWARD"=2] ("Readout Direction")
                w683 = u32 4212128 items=["SENSOR MODE"=4212128, "CCD MODE"=4212384, "READOUT MODE"=4211872, "ACTIVE VIEW INDEX"=4343136, "BITS PER CHANNEL"=4342976, "IMAGE PIXEL TYPE"=4343296, "BINNING"=4215968, "EXPOSURE TIME"=2049184, "CONTRAST GAIN"=3163312, "CONTRAST OFFSET"=3163328, "LIGHT MODE"=2114720, "SENSITIVITY"=2114992, "PHOTON IMAGING MODE"=2115200, "HIGH DYNAMIC RANGE MODE"=3163360, "WHITE BALANCE"=3163568, "TEMPERATURE"=2115232, "TEMPERATURE TARGET"=2115264, "SENSOR COOLER FAN"=2115296, "LINEBUNDLE HEIGHT"=4212192, "MECHANICAL SHUTTER"=2115488, "BACK FOCUS POSITION"=8422304, "TRIGGER CONNECTOR"=1066432, "TRIGGER SOURCE"=1066144, "OUTPUT TRIGGER SOURCE"=1852576, "TRIGGER GLOBAL EXPOSURE"=2049680, "FIRST TRIGGER BEHAVIOR"=2049696, "CHANNEL SYNC"=1852352, "READOUT DIRECTION"=4211904, "PRE HSYNC COUNT"=1852704, "INTERNAL LINE SPEED"=4191408, "INTERNAL LINE INTERVAL"=4191424] ("Parameter")
                w682 = u32 4211904 items=["SENSOR MODE"=4212128, "CCD MODE"=4212384, "READOUT MODE"=4211872, "ACTIVE VIEW INDEX"=4343136, "BITS PER CHANNEL"=4342976, "IMAGE PIXEL TYPE"=4343296, "BINNING"=4215968, "EXPOSURE TIME"=2049184, "CONTRAST GAIN"=3163312, "CONTRAST OFFSET"=3163328, "LIGHT MODE"=2114720, "SENSITIVITY"=2114992, "PHOTON IMAGING MODE"=2115200, "HIGH DYNAMIC RANGE MODE"=3163360, "WHITE BALANCE"=3163568, "TEMPERATURE"=2115232, "TEMPERATURE TARGET"=2115264, "SENSOR COOLER FAN"=2115296, "LINEBUNDLE HEIGHT"=4212192, "MECHANICAL SHUTTER"=2115488, "BACK FOCUS POSITION"=8422304, "TRIGGER CONNECTOR"=1066432, "TRIGGER SOURCE"=1066144, "OUTPUT TRIGGER SOURCE"=1852576, "TRIGGER GLOBAL EXPOSURE"=2049680, "FIRST TRIGGER BEHAVIOR"=2049696, "CHANNEL SYNC"=1852352, "READOUT DIRECTION"=4211904, "PRE HSYNC COUNT"=1852704, "INTERNAL LINE SPEED"=4191408, "INTERNAL LINE INTERVAL"=4191424] ("Parameter")
                n131 = case shown="\"Master\"" enum16{"Master", "Slave"}."Master" ("Camera Trigger Mode") {
                  tunnel: [w694 w710] -> w681
                  tunnel: [w693 w708] -> w680
                  tunnel: w676 -> [w692 w712]
                  tunnel: w675 -> [w691 w711]
                  frame "Slave", Default {
                    w699 = u32 2 items=["NEGATIVE"=1, "POSITIVE"=2] ("Input Trigger Polarity")
                    w698 = u32 2 items=["INTERNAL"=1, "EXTERNAL EDGE"=2, "EXTERNAL LEVEL"=4, "SOFTWARE"=32, "FAST REPETITION"=64, "TDI"=128, "START"=512, "SYNC READOUT"=1024] ("Input Trigger Mode")
                    n132 = Bundle("Input Trigger Mode"=w698, "Input Trigger Polarity"=w699, "Times"=u32 1, "Delay"=0.0) -> (w695:T13)  [unwired: 1 in]
                    n133 = call <userlib>:"tm_setinputtrigger_40.vi"("error in (no error)"=w691, "Parameters"=w695, "Handle in"=w692) -> ("error out"=w693:errorcluster, "Handle out"=w694:u32)  [unwired: 7 in]
                  }
                  frame "Master" {
                    w705 = u32 2 items=["Exposure"=1, "Readout End"=2, "V Sync"=3, "H Sync"=4, "Trigger"=6] ("Source")
                    w707 = u32 2 items=["NEGATIVE"=1, "POSITIVE"=2] ("Output Trigger Polarity")
                    w706 = u32 3 items=["LOW"=1, "GLOBAL EXPOSURE"=2, "PROGRAMMABLE"=3, "TRIGGER READY"=4, "HIGH"=5] ("Output Trigger Mode")
                    w718 = u32 2 items=["NEGATIVE"=1, "POSITIVE"=2] ("Input Trigger Polarity")
                    w717 = u32 1 items=["INTERNAL"=1, "EXTERNAL EDGE"=2, "EXTERNAL LEVEL"=4, "SOFTWARE"=32, "FAST REPETITION"=64, "TDI"=128, "START"=512, "SYNC READOUT"=1024] ("Input Trigger Mode")
                    n134 = Bundle("Input Trigger Mode"=w717, "Input Trigger Polarity"=w718, "Times"=u32 1, "Delay"=0.0) -> (w714:T13)  [unwired: 1 in]
                    n135 = call <userlib>:"tm_setinputtrigger_40.vi"("error in (no error)"=w711, "Parameters"=w714, "Handle in"=w712) -> ("error out"=w709:errorcluster, "Handle out"=w713:u32)  [unwired: 7 in]
                    n136 = Bundle("Output Trigger Period"=0.001, "Delay"=0.0, "Source"=w705) -> (w702:T14)  [unwired: 1 in]
                    n137 = Bundle("Output Trigger Mode"=w706, "Output Trigger Polarity"=w707) -> (w701:T15)  [unwired: 1 in]
                    n138 = call <userlib>:"tm_setoutputtrigger_40.vi"("Port"=1, "error in (no error)"=w709, "Programmable Options"=w702, "Type"=w701, "Handle in"=w713) -> ("error out"=w708:errorcluster, "Handle out"=w710:u32)  [unwired: 5 in]
                  }
                }
                n139 = Bundle By Name(cluster=w687, "Received?"=TRUE ("Running?"), "Camera Actions"=Orca_Flash_Actions."IDLE") -> (w686:T6)
                n140 = call <userlib>:"tm_setparameter_40.vi"("error in (no error)"=w680, "Value in"=12.0, "Parameter"=w683, "Handle in"=w681) -> ("error out"=w685:errorcluster, "Handle out"=w684:u32)  [unwired: 6 in]
                n141 = To Double Precision Float(number=w679) -> (double precision float=w678:dbl)
                n142 = call <userlib>:"tm_setparameter_40.vi"("error in (no error)"=w685, "Value in"=w678, "Parameter"=w682, "Handle in"=w684) -> ("error out"=w673:errorcluster, "Handle out"=w674:u32)  [unwired: 6 in]
                n143 = call <userlib>:"tm_setparameter_40.vi"("error in (no error)"=w673, "Value in"="Internal Line Interval Setpoint", "Parameter"=w668, "Handle in"=w674) -> ("error out"=w671:errorcluster, "Handle out"=w672:u32)  [unwired: 6 in]
                n144 = call <userlib>:"tm_getparameter_40.vi"("error in (no error)"=w671, "Parameter"=w668, "Handle in"=w672) -> ("error out"=w669:errorcluster, "Value out"=w666:dbl, "Handle out"=w670:u32)  [unwired: 6 in]
                n145 = Multiply(x=w666, y="Number of lines") -> (x*y=w665:dbl)
                n146 = call <userlib>:"tm_setparameter_40.vi"("error in (no error)"=w669, "Value in"=w665, "Parameter"=w662, "Handle in"=w670) -> ("error out"=w663:errorcluster)  [unwired: 6 in, 1 out]
              }
              frame "AREA MODE" {
                w723 = u32 2049184 items=["SENSOR MODE"=4212128, "READOUT SPEED"=4211872, "READOUT DIRECTION"=4211904, "TRIGGER GLOBAL EXPOSURE"=2049680, "TRIGGER DELAY"=1066480, "INTERNAL TRIGGER HANDLING"=1066496, "SYNC READOUT SYSTEM BLANK"=1066528, "SENSOR TEMPERATURE"=2115232, "SENSOR COOLER STATUS"=2115280, "EXPOSURE TIME"=2049184, "DEFECT CORRECT MODE"=4670368, "BINNING"=4215968, "INTERNAL LINE SPEED"=4226000, "INTERNAL LINE INTERVAL"=4226016, "NUMBER OF OUTPUT TRIGGER CONNECTOR"=1852320, "OUTPUT TRIGGER SOURCE[0]"=1852576, "OUTPUT TRIGGER SOURCE[1]"=1852832, "OUTPUT TRIGGER SOURCE[2]"=1853088, "OUTPUT TRIGGER POLARITY[0]"=1852592, "OUTPUT TRIGGER POLARITY[1]"=1852848, "OUTPUT TRIGGER POLARITY[2]"=1853104, "OUTPUT TRIGGER ACTIVE[0]"=1852608, "OUTPUT TRIGGER ACTIVE[1]"=1852864, "OUTPUT TRIGGER ACTIVE[2]"=1853120, "OUTPUT TRIGGER DELAY[0]"=1852624, "OUTPUT TRIGGER DELAY[1]"=1852880, "OUTPUT TRIGGER DELAY[2]"=1853136, "OUTPUT TRIGGER PERIOD[0]"=1852640, "OUTPUT TRIGGER PERIOD[1]"=1852896, "OUTPUT TRIGGER PERIOD[2]"=1853152, "OUTPUT TRIGGER KIND[0]"=1852656, "OUTPUT TRIGGER KIND[1]"=1852912, "OUTPUT TRIGGER KIND[2]"=1853168, "OUTPUT TRIGGER BASE SENSOR[0]"=1852672, "OUTPUT TRIGGER BASE SENSOR[1]"=1852928, "OUTPUT TRIGGER BASE SENSOR[2]"=1853184, "OUTPUT TRIGGER PRE HSYNC COUNT"=1852704] ("Parameter")
                w724 = u32 2 items=["NEGATIVE"=1, "POSITIVE"=2] ("Input Trigger Polarity")
                w738 = u32 1 items=["INTERNAL"=1, "EXTERNAL EDGE"=2, "EXTERNAL LEVEL"=4, "SOFTWARE"=32, "FAST REPETITION"=64, "TDI"=128, "START"=512, "SYNC READOUT"=1024] ("Input Trigger Mode")
                w734 = u32 4212128 items=["SENSOR MODE"=4212128, "CCD MODE"=4212384, "READOUT MODE"=4211872, "ACTIVE VIEW INDEX"=4343136, "BITS PER CHANNEL"=4342976, "IMAGE PIXEL TYPE"=4343296, "BINNING"=4215968, "EXPOSURE TIME"=2049184, "CONTRAST GAIN"=3163312, "CONTRAST OFFSET"=3163328, "LIGHT MODE"=2114720, "SENSITIVITY"=2114992, "PHOTON IMAGING MODE"=2115200, "HIGH DYNAMIC RANGE MODE"=3163360, "WHITE BALANCE"=3163568, "TEMPERATURE"=2115232, "TEMPERATURE TARGET"=2115264, "SENSOR COOLER FAN"=2115296, "LINEBUNDLE HEIGHT"=4212192, "MECHANICAL SHUTTER"=2115488, "BACK FOCUS POSITION"=8422304, "TRIGGER CONNECTOR"=1066432, "TRIGGER SOURCE"=1066144, "OUTPUT TRIGGER SOURCE"=1852576, "TRIGGER GLOBAL EXPOSURE"=2049680, "FIRST TRIGGER BEHAVIOR"=2049696, "CHANNEL SYNC"=1852352, "READOUT DIRECTION"=4211904, "PRE HSYNC COUNT"=1852704, "INTERNAL LINE SPEED"=4191408, "INTERNAL LINE INTERVAL"=4191424] ("Parameter")
                n147 = Bundle("Input Trigger Mode"=w738, "Input Trigger Polarity"=w724, "Times"=u32 1, "Delay"=0.0) -> (w735:T13)  [unwired: 1 in]
                n148 = call <userlib>:"tm_setinputtrigger_40.vi"("error in (no error)"=w729, "Parameters"=w735, "Handle in"=w730) -> ("error out"=w732:errorcluster, "Handle out"=w733:u32)  [unwired: 7 in]
                n149 = Bundle By Name(cluster=w726, "Received?"=TRUE ("Running?"), "Camera Actions"=Orca_Flash_Actions."IDLE") -> (w725:T6)
                n150 = call <userlib>:"tm_setparameter_40.vi"("error in (no error)"=w732, "Value in"=1.0, "Parameter"=w734, "Handle in"=w733) -> ("error out"=w720:errorcluster, "Handle out"=w721:u32)  [unwired: 6 in]
                n151 = call <userlib>:"tm_setparameter_40.vi"("error in (no error)"=w720, "Value in"=0.1, "Parameter"=w723, "Handle in"=w721) -> ("error out"=w719:errorcluster)  [unwired: 6 in, 1 out]
              }
            }
            n152 = Send Notification(notification=w327, notifier=w330) -> (notifier out=w323:refnum<notifier>)  [unwired: 1 in, 1 out]
          }
          frame Error {
            n153 = Unbundle By Name(w741) -> ("source"=w742:string)
            n154 = call <vilib>:"Space Constant.vi"() -> ("String"=w745:string)
            n155 = Concatenate Strings(w740, w745, "Device Error." ("string"), "\r", w742) -> (w746:string)
            n156 = One Button Dialog(message=w746) -> ()  [unwired: 1 in, 1 out]
          }
        }
      }
      n157 = while {
        tunnel: w37 -> [w47]
        tunnel: w41 -> [w46]
        tunnel: w34 -> [w45]
        stop <- w49 stop-if-true
        n158 = event shown="[0] Timeout" {
          selector: _ -> [_ _ _ _ _ _ _ _]
          dyn-events: _ -> [_ _ _ _ _ _ _ _]
          timeout: 200 -> [_ _ _ _ _ _ _ _]
          tunnel: w47 -> [w62 _ w93 w131 w174 w222 w246 w290]
          tunnel: [w58 FALSE ("NewVal") FALSE ("NewVal") FALSE ("NewVal") FALSE ("NewVal") FALSE ("NewVal") FALSE ("NewVal") w294] -> w49
          tunnel: w46 -> [w55 _ _ _ _ _ _ _]
          tunnel: w45 -> [w54 _ _ _ _ _ _ _]
          event Timeout {
            n159 = event-data() -> ()  [unwired: 1 in, 1 out]
            n160 = call "Common Device Queue Get Command.vi"("Common Queue"=w55, "Notifier Name"=w54) -> ("Command"=w57:string)  [unwired: 12 in, 1 out]
            n161 = Get Notifier Status(notifier=w62) -> (notifier out=w52:refnum<notifier>, current notification=w61:T6, error out=w60:errorcluster)  [unwired: 1 in, 2 out]
            n162 = control-ref of="This VI"() -> (w56:refnum<vi>)
            n163 = Unbundle By Name(w61) -> ("Running?"=w51:bool, "bead collection"=→"bead collection":bool)
            n164 = Unbundle By Name(w60) -> ("status"=w59:bool)
            n165 = call "Common Device Queue Execute Command.vi"("Common Command"=w57, "VI Refnum"=w56) -> ("Quit?"=w53:bool)  [unwired: 12 in, 1 out]
            n166 = disable-structure shown="Enabled" {
              disable-tunnel: w51 -> [w63 _]
              frame Disabled {
                n167 = case shown="False" w63 {
                  frame False {
                    w64 = FALSE ("RECORD")
                    n168 = local write "PREVIEW"(w64) -> ()
                    n169 = local write "RECORD"(w64) -> ()
                  }
                  frame True {
                  }
                }
              }
              frame Enabled {
              }
            }
            n170 = Or(x=w53, y=w59) -> (x .or. y?=w58:bool)
            n171 = case shown="True" w53 {
              tunnel: w52 -> [_ w75]
              frame False {
              }
              frame True {
                n172 = Get Notifier Status(notifier=w75) -> (notifier out=w72:refnum<notifier>, current notification=w74:T6)  [unwired: 1 in, 3 out]
                n173 = Bundle By Name(cluster=w74, "Running?"=FALSE) -> (w71:T6)
                n174 = Send Notification(notification=w71, notifier=w72) -> (notifier out=w69:refnum<notifier>)  [unwired: 1 in, 1 out]
                n175 = for {
                  N: 5000 -> [_]
                  tunnel: w69 -> [w80]
                  tunnel: [w78] -> w68
                  tunnel: [w76] -> w67
                  stop <- w79 stop-if-true
                  n176 = Get Notifier Status(notifier=w80) -> (notifier out=w78:refnum<notifier>, current notification=w76:T6, # waiting=w81:i32)  [unwired: 1 in, 2 out]
                  n177 = Wait (ms)(milliseconds to wait=u32 1) -> ()  [unwired: 1 out]
                  n178 = Greater Than 0?(x=w81) -> (x > 0?=w79:bool)
                }
                n179 = Bundle By Name(cluster=w67, "Camera Actions"=Orca_Flash_Actions."QUIT") -> (w65:T6)
                n180 = Send Notification(notification=w65, notifier=w68) -> ()  [unwired: 1 in, 2 out]
              }
            }
          }
          event Application Instance Close? {
            n181 = event-data() -> ()  [unwired: 1 in, 5 out]
            n182 = control-ref of="This VI"() -> (w84:refnum<vi>)
            n183 = invoke class="VI" method="FP.Open"(reference=w84, "Activate"=TRUE ("Activate?"), "State"=T9."Standard") -> ()  [unwired: 2 in, 5 out]
            n184 = event-data("Discard?"=TRUE) -> ()  [unwired: 1 in, 1 out]
          }
          event "Set ROI", "Get ROI": Value Change {
            n185 = event-data() -> ("CtlRef"=w103:refnum<vi>)  [unwired: 1 in, 1 out]
            n186 = Get Notifier Status(notifier=w93) -> (notifier out=w91:refnum<notifier>, current notification=w90:T6, # waiting=w89:i32)  [unwired: 1 in, 2 out]
            n187 = Equal To 0?(x=w89) -> (x = 0?=w92:bool)
            n188 = case shown="True" w92 {
              tunnel: [w107 w113] -> w95
              tunnel: [w106 w112] -> w94
              tunnel: w91 -> [w107 w111]
              tunnel: w90 -> [w106 w108]
              frame False {
              }
              frame True {
                n189 = Bundle By Name(cluster=w108, "Running?"=FALSE, "Camera Actions"=Orca_Flash_Actions."IDLE") -> (w115:T6)
                n190 = Send Notification(notification=w115, notifier=w111) -> (notifier out=w116:refnum<notifier>)  [unwired: 1 in, 1 out]
                n191 = for {
                  N: 2000 -> [_]
                  tunnel: w116 -> [w122]
                  tunnel: [w119] -> w113
                  tunnel: [w118] -> w112
                  stop <- w120 stop-if-true
                  n192 = Get Notifier Status(notifier=w122) -> (notifier out=w119:refnum<notifier>, current notification=w118:T6, # waiting=w121:i32)  [unwired: 1 in, 2 out]
                  n193 = Not Equal To 0?(x=w121) -> (x != 0?=w120:bool)
                  n194 = Wait (ms)(milliseconds to wait=u32 1) -> ()  [unwired: 1 out]
                }
              }
            }
            n195 = property class="Bool"(reference=w103) -> ("Label.Text"=w102:string)  [unwired: 1 in, 2 out]
            n196 = case shown="\"Get ROI\", Default" w102 {
              tunnel: [Orca_Flash_Actions."GETROI" ("Camera Actions") Orca_Flash_Actions."SETROI" ("Camera Actions")] -> w101
              tunnel: [w123 w125] -> w100
              tunnel: "Orca Flash ROI" -> [w123 w125]
              frame "Get ROI", Default {
              }
              frame "Set ROI" {
              }
            }
            n197 = Bundle By Name(cluster=w94, "Running?"=FALSE, "Camera Actions"=w101, "sCMOS ROI"=w100) -> (w99:T6)
            n198 = Send Notification(notification=w99, notifier=w95) -> (notifier out=w98:refnum<notifier>)  [unwired: 1 in, 1 out]
            n199 = Wait on Notification(notifier=w98, ignore previous (F)=TRUE) -> (notification=w97:T6)  [unwired: 2 in, 3 out]
            n200 = Unbundle By Name(w97) -> ("sCMOS ROI"=w87:T1)
            n201 = local write "Orca Flash ROI"(w87) -> ()
          }
          event "Set Parameter", "Get Parameter": Value Change {
            n202 = event-data() -> ("CtlRef"=w142:refnum<vi>)  [unwired: 1 in, 1 out]
            n203 = Get Notifier Status(notifier=w131) -> (notifier out=w129:refnum<notifier>, current notification=w128:T6, # waiting=w127:i32)  [unwired: 1 in, 2 out]
            n204 = Equal To 0?(x=w127) -> (x = 0?=w130:bool)
            n205 = case shown="True" w130 {
              tunnel: w129 -> [w146 w155]
              tunnel: w128 -> [w145 w154]
              tunnel: [w146 w150] -> w134
              tunnel: [w145 w149] -> w133
              frame False {
              }
              frame True {
                n206 = Bundle By Name(cluster=w154, "Running?"=FALSE, "Camera Actions"=Orca_Flash_Actions."IDLE") -> (w152:T6)
                n207 = Send Notification(notification=w152, notifier=w155) -> (notifier out=w151:refnum<notifier>)  [unwired: 1 in, 1 out]
                n208 = for {
                  N: 2000 -> [_]
                  tunnel: w151 -> [w161]
                  tunnel: [w158] -> w150
                  tunnel: [w157] -> w149
                  stop <- w159 stop-if-true
                  n209 = Get Notifier Status(notifier=w161) -> (notifier out=w158:refnum<notifier>, current notification=w157:T6, # waiting=w160:i32)  [unwired: 1 in, 2 out]
                  n210 = Not Equal To 0?(x=w160) -> (x != 0?=w159:bool)
                  n211 = Wait (ms)(milliseconds to wait=u32 1) -> ()  [unwired: 1 out]
                }
              }
            }
            n212 = property class="Bool"(reference=w142) -> ("Label.Text"=w141:string)  [unwired: 1 in, 2 out]
            n213 = case shown="\"Set Parameter\"" w141 {
              tunnel: [Orca_Flash_Actions."GETPARAM" ("Camera Actions") Orca_Flash_Actions."SETPARAM" ("Camera Actions")] -> w140
              frame "Get Parameter", Default {
              }
              frame "Set Parameter" {
              }
            }
            n214 = Bundle By Name(cluster=w133, "sCMOS Parameter"="sCMOS Parameter", "Running?"=FALSE, "Camera Actions"=w140) -> (w139:T6)
            n215 = Send Notification(notification=w139, notifier=w134) -> (notifier out=w138:refnum<notifier>)  [unwired: 1 in, 1 out]
            n216 = Wait on Notification(notifier=w138, ignore previous (F)=TRUE) -> (notification=w137:T6)  [unwired: 2 in, 3 out]
            n217 = Unbundle By Name(w137) -> ("sCMOS Parameter"=w136:T2)
            n218 = local write "sCMOS Parameter"(w136) -> ()
          }
          event "PREVIEW", "RECORD": Value Change {
            n219 = event-data() -> ("CtlRef"=w178:refnum<vi>, "NewVal"=w176:bool)  [unwired: 1 in, 1 out]
            n220 = Get Notifier Status(notifier=w174) -> (notifier out=w166:refnum<notifier>, current notification=w165:T6, # waiting=w164:i32)  [unwired: 1 in, 2 out]
            n221 = Equal To 0?(x=w164) -> (x = 0?=w167:bool)
            n222 = property class="Bool (strict)"(reference=w178) -> ("Label.Text"=w177:string)  [unwired: 1 in, 2 out]
            n223 = case shown="True" w167 {
              tunnel: w166 -> [w199 w208]
              tunnel: [w199 w204] -> w169
              tunnel: [w198 w202] -> w168
              tunnel: w165 -> [w198 w201]
              frame False {
              }
              frame True {
                n224 = Bundle By Name(cluster=w201, "Running?"=FALSE, "Camera Actions"=Orca_Flash_Actions."IDLE") -> (w206:T6)
                n225 = Send Notification(notification=w206, notifier=w208) -> (notifier out=w205:refnum<notifier>)  [unwired: 1 in, 1 out]
                n226 = for {
                  N: 2000 -> [_]
                  tunnel: w205 -> [w214]
                  tunnel: [w213] -> w204
                  tunnel: [w212] -> w202
                  stop <- w210 stop-if-true
                  n227 = Get Notifier Status(notifier=w214) -> (notifier out=w213:refnum<notifier>, current notification=w212:T6, # waiting=w211:i32)  [unwired: 1 in, 2 out]
                  n228 = Not Equal To 0?(x=w211) -> (x != 0?=w210:bool)
                  n229 = Wait (ms)(milliseconds to wait=u32 1) -> ()  [unwired: 1 out]
                }
              }
            }
            n230 = case shown="\"PREVIEW\"" w177 {
              tunnel: w176 -> [w182 _ w192]
              tunnel: [w181 FALSE w191] -> w172
              tunnel: [w180 Orca_Flash_Actions."IDLE" ("Camera Actions") w190] -> w175
              frame "PREVIEW" {
                n231 = case shown="False" w182 {
                  selector: w182 -> [_ w187]
                  tunnel: [FALSE w186] -> w181
                  tunnel: [Orca_Flash_Actions."IDLE" ("Camera Actions") Orca_Flash_Actions."PREVIEW" ("Camera Actions")] -> w180
                  frame False {
                  }
                  frame True {
                    n232 = Not(x=w187) -> (.not. x?=w186:bool)
                    n233 = local write "RECORD"(w186) -> ()
                  }
                }
              }
              frame Default {
              }
              frame "RECORD" {
                n234 = case shown="True" w192 {
                  selector: w192 -> [_ w197]
                  tunnel: [FALSE w196] -> w191
                  tunnel: [Orca_Flash_Actions."IDLE" ("Camera Actions") Orca_Flash_Actions."RECORD" ("Camera Actions")] -> w190
                  frame False {
                  }
                  frame True {
                    n235 = Not(x=w197) -> (.not. x?=w196:bool)
                    n236 = local write "PREVIEW"(w196) -> ()
                  }
                }
              }
            }
            n237 = Bundle By Name(cluster=w168, "# of frames"="# of frames", "Save Path"="Path", "Running?"=w172, "Camera Actions"=w175) -> (w173:T6)
            n238 = Send Notification(notification=w173, notifier=w169) -> ()  [unwired: 1 in, 2 out]
          }
          event "Sensor Mode", "Internal Line Interval Setpoint", "Number of lines": Value Change {
            n239 = event-data() -> ()  [unwired: 1 in, 6 out]
            n240 = Get Notifier Status(notifier=w222) -> (notifier out=w225:refnum<notifier>, current notification=w224:T6, # waiting=w223:i32)  [unwired: 1 in, 2 out]
            n241 = Equal To 0?(x=w223) -> (x = 0?=w226:bool)
            n242 = case shown="True" w226 {
              tunnel: w225 -> [w230 w239]
              tunnel: w224 -> [w229 w238]
              tunnel: [w230 w234] -> w221
              tunnel: [w229 w233] -> w220
              frame False {
              }
              frame True {
                n243 = Bundle By Name(cluster=w238, "Running?"=FALSE, "Camera Actions"=Orca_Flash_Actions."IDLE") -> (w236:T6)
                n244 = Send Notification(notification=w236, notifier=w239) -> (notifier out=w235:refnum<notifier>)  [unwired: 1 in, 1 out]
                n245 = for {
                  N: 2000 -> [_]
                  tunnel: w235 -> [w245]
                  tunnel: [w242] -> w234
                  tunnel: [w241] -> w233
                  stop <- w243 stop-if-true
                  n246 = Get Notifier Status(notifier=w245) -> (notifier out=w242:refnum<notifier>, current notification=w241:T6, # waiting=w244:i32)  [unwired: 1 in, 2 out]
                  n247 = Not Equal To 0?(x=w244) -> (x != 0?=w243:bool)
                  n248 = Wait (ms)(milliseconds to wait=u32 1) -> ()  [unwired: 1 out]
                }
              }
            }
            n249 = case shown="\"Progressive\"" "Sensor Mode" {
              tunnel: [Orca_Flash_Actions."AREA MODE" ("Camera Actions") Orca_Flash_Actions."PROGRESSIVE MODE" ("Camera Actions")] -> w216
              frame "Area", Default {
              }
              frame "Progressive" {
              }
            }
            n250 = Bundle By Name(cluster=w220, "Running?"=FALSE, "Camera Actions"=w216) -> (w215:T6)
            n251 = Send Notification(notification=w215, notifier=w221) -> ()  [unwired: 1 in, 2 out]
          }
          event "Use Display Module": Value Change {
            n252 = event-data() -> ("NewVal"=w247:bool)  [unwired: 1 in]
            n253 = Get Notifier Status(notifier=w246) -> (current notification=w248:T6)  [unwired: 1 in, 4 out]
            n254 = Unbundle By Name(w248) -> ("Image Ref"=w262:T8)
            n255 = Obtain Notifier(name (unnamed)="Display Module IMAQ Refs", notification data type=T8[] [], create if not found? (T)=FALSE) -> (notifier out=w255:refnum<notifier>, error out=w256:errorcluster)  [unwired: 1 in, 1 out]
            n256 = Get Notifier Status(notifier=w255, error in (no error)=w256) -> (notifier out=w254:refnum<notifier>, current notification=w252:T8[], error out=w253:errorcluster)  [unwired: 2 out]
            n257 = case shown="False" w247 {
              tunnel: w254 -> [w271 w281]
              tunnel: w253 -> [w265 w280]
              tunnel: w252 -> [w267 w283]
              tunnel: [w266 w282] -> w249
              tunnel: [w271 w281] -> w251
              tunnel: [w265 w280] -> w250
              tunnel: w262 -> [w264 w279]
              frame False {
                n258 = Equal?(x=w267, y=w264) -> (x = y?=w270:bool[])
                n259 = for {
                  tunnel: w270 -> [w278] mode=indexing
                  tunnel: [w277] -> w268
                  i -> [w277]
                  stop <- w278 stop-if-true
                }
                n260 = Or Array Elements(Boolean array=w270) -> (logical OR=w269:bool)
                n261 = case shown="True" w269 {
                  tunnel: w268 -> [_ w275]
                  tunnel: w267 -> [w272 w274]
                  tunnel: [w272 w273] -> w266
                  frame False {
                  }
                  frame True {
                    n262 = Delete From Array(array=w274, length=1, index=w275) -> (array with subset deleted=w273:T8[])  [unwired: 1 out]
                  }
                }
              }
              frame True {
                n263 = Build Array (concatenate)(w283, w279) -> (w282:T8[])
              }
            }
            n264 = Send Notification(notification=w249, notifier=w251, error in (no error)=w250) -> (notifier out=w257:refnum<notifier>, error out=w258:errorcluster)
            n265 = Release Notifier(notifier=w257, error in (no error)=w258) -> ()  [unwired: 1 in, 3 out]
          }
          event "QUIT": Value Change {
            n266 = event-data() -> ("NewVal"=w294:bool)  [unwired: 1 in]
            n267 = Get Notifier Status(notifier=w290) -> (notifier out=w286:refnum<notifier>, current notification=w285:T6, # waiting=w284:i32)  [unwired: 1 in, 2 out]
            n268 = Equal To 0?(x=w284) -> (x = 0?=w287:bool)
            n269 = case shown="True" w287 {
              tunnel: w286 -> [w296 w301]
              tunnel: [w296 w299] -> w289
              tunnel: [w295 w298] -> w288
              tunnel: w285 -> [w295 w297]
              frame False {
              }
              frame True {
                n270 = Bundle By Name(cluster=w297, "Running?"=FALSE, "Camera Actions"=Orca_Flash_Actions."IDLE") -> (w300:T6)
                n271 = Send Notification(notification=w300, notifier=w301) -> (notifier out=w304:refnum<notifier>)  [unwired: 1 in, 1 out]
                n272 = for {
                  N: 2000 -> [_]
                  tunnel: w304 -> [w311]
                  tunnel: [w308] -> w299
                  tunnel: [w307] -> w298
                  stop <- w309 stop-if-true
                  n273 = Get Notifier Status(notifier=w311) -> (notifier out=w308:refnum<notifier>, current notification=w307:T6, # waiting=w310:i32)  [unwired: 1 in, 2 out]
                  n274 = Not Equal To 0?(x=w310) -> (x != 0?=w309:bool)
                  n275 = Wait (ms)(milliseconds to wait=u32 1) -> ()  [unwired: 1 out]
                }
              }
            }
            n276 = Bundle By Name(cluster=w288, "Running?"=FALSE, "Camera Actions"=Orca_Flash_Actions."QUIT") -> (w293:T6)
            n277 = Send Notification(notification=w293, notifier=w289) -> ()  [unwired: 1 in, 2 out]
          }
        }
      }
      n278 = Release Notifier(notifier=w35, force destroy? (F)=TRUE) -> ()  [unwired: 1 in, 3 out]
    }
    frame Error {
      n279 = call <userlib>:"tm_deinitialize_40.vi"("error in (no error)"=w760) -> ("error out"=w752:errorcluster)  [unwired: 10 in]
      n280 = Release Notifier(notifier=w753, force destroy? (F)=TRUE, error in (no error)=w752) -> (error out=w751:errorcluster)  [unwired: 2 out]
      n281 = Unbundle By Name(w751) -> ("source"=w755:string)
      n282 = call <vilib>:"Space Constant.vi"() -> ("String"=w758:string)
      n283 = Concatenate Strings(w750, w758, "Device Error." ("string"), "\r", w755) -> (w759:string)
      n284 = One Button Dialog(message=w759) -> ()  [unwired: 1 in, 1 out]
    }
  }
